vi "Share in Browser.vi"   [LabVIEW 2020]
doc: "Tools menu entry Tools > RemoteVI > Share in Browser (installed by the VIPM package into <LabVIEW>\\project\\RemoteVI): opens RemoteVI Server (RemoteVI Open Server.vi) and closes its own window again."
uses:
  source/RemoteVI.lvlib
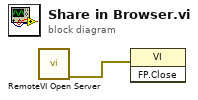
[diagram p0: block diagram]
diagram:
  n1 = call "RemoteVI Open Server.vi"() -> ("error out"=w1:errorcluster)  [unwired: 15 in]
  n2 = invoke class="VI" method="FP.Close"(error in=w1) -> ()  [unwired: 2 in, 3 out]
